vi "SDO_TRAJECTORY_EXECUTE_REL.vi"(6 "EnableClosedLoop":bool=TRUE, 8 "Init":bool, 10 "End Relative\nOrientation Deg":dbl, 11 "Gyro Heading\nRAD":dbl) -> (0 "AtReference":bool, 3 "Chassis Velocity Target":T1 {"vOmega" format="%10.3f"; "vY" format="%10.3f"; "vX" format="%10.3f"})   [LabVIEW 2019]
uses:
  <vilib>/Rock Robotics/WPI/ThirdParty/JAS_Junk/TrajLib/TypeDef/CHASSIS_SPEEDS.ctl
  <vilib>/Rock Robotics/WPI/ThirdParty/JAS_Junk/TrajLib/VI/Util_GetTime_U32.vi
  <vilib>/Rock Robotics/WPI/ThirdParty/JAS_Junk/TrajLib/ProfiledPIDController_NewPeriod.vi
  <vilib>/Rock Robotics/WPI/ThirdParty/JAS_Junk/TrajLib/ProfiledPIDController_SetIntegratorRange.vi
  <vilib>/Rock Robotics/WPI/ThirdParty/JAS_Junk/TrajLib/ProfiledPIDController_DisableContInput.vi
  <vilib>/Rock Robotics/WPI/ThirdParty/JAS_Junk/TrajLib/ProfiledPIDController_EnableContInput.vi
  <vilib>/Rock Robotics/WPI/ThirdParty/JAS_Junk/TrajLib/TrapProfConstraint_New.vi
  <vilib>/Rock Robotics/WPI/ThirdParty/JAS_Junk/TrajLib/Conv_Deg_Radians.vi
  <vilib>/Rock Robotics/WPI/ThirdParty/JAS_Junk/TrajLib/Translation2d_Create.vi
  <vilib>/Rock Robotics/WPI/ThirdParty/JAS_Junk/TrajLib/SwerveOdometry_UpdateX.vi
  <vilib>/Rock Robotics/WPI/ThirdParty/JAS_Junk/TrajLib/SwerveOdometry_ResetPosition.vi
  <vilib>/Rock Robotics/WPI/ThirdParty/JAS_Junk/TrajLib/SwerveOdometry_New.vi
  <vilib>/Rock Robotics/WPI/ThirdParty/JAS_Junk/TrajLib/HolDrvCtrl_New.vi
  <vilib>/Rock Robotics/WPI/ThirdParty/JAS_Junk/TrajLib/HolDrvCtrl_PackPID.vi
  <vilib>/Rock Robotics/WPI/ThirdParty/JAS_Junk/TrajLib/HolDrvCtrl_SetTolerance.vi
  <vilib>/Rock Robotics/WPI/ThirdParty/JAS_Junk/TrajLib/HolDrvCtrl_SetEnabled.vi
  <vilib>/Rock Robotics/WPI/ThirdParty/JAS_Junk/TrajLib/HolDrvCtrl_Calculate_Trajectory.vi
  <vilib>/Rock Robotics/WPI/ThirdParty/JAS_Junk/TrajLib/HolDrvCtrl_AtReference.vi
  <vilib>/Rock Robotics/WPI/ThirdParty/JAS_Junk/TrajLib/TrapProfState_New.vi
  <vilib>/Rock Robotics/WPI/ThirdParty/JAS_Junk/TrajLib/PIDController_NewPeriod.vi
  <vilib>/Rock Robotics/SystemInterfaces/NetworkCommunication/NetComm_UsageReport_report.vi
  <vilib>/Rock Robotics/WPI/ThirdParty/JAS_Junk/TrajLib/PIDController_SetIntegratorRange.vi
  <vilib>/Rock Robotics/WPI/ThirdParty/JAS_Junk/TrajLib/PIDController_DisableContinousInput.vi
  <vilib>/Rock Robotics/WPI/ThirdParty/JAS_Junk/TrajLib/PIDController_EnableContinousInput.vi
  <vilib>/Rock Robotics/WPI/ThirdParty/JAS_Junk/TrajLib/Rotation2d_Plus.vi
  <vilib>/Rock Robotics/WPI/ThirdParty/JAS_Junk/TrajLib/Twist2d_Create.vi
  <vilib>/Rock Robotics/WPI/ThirdParty/JAS_Junk/TrajLib/Rotation2d_Minus.vi
  <vilib>/Rock Robotics/WPI/ThirdParty/JAS_Junk/TrajLib/Pose2d_getTranslation.vi
  <vilib>/Rock Robotics/WPI/ThirdParty/JAS_Junk/TrajLib/Pose2d_New_TRRO.vi
  <vilib>/Rock Robotics/WPI/ThirdParty/JAS_Junk/TrajLib/VI/SwerveModulePosition_Get.vi
  <vilib>/Rock Robotics/WPI/ThirdParty/JAS_Junk/TrajLib/VI/SwerveModulePosition_New.vi
  <vilib>/Rock Robotics/WPI/ThirdParty/JAS_Junk/TrajLib/Twist2d_GetAll.vi
  <vilib>/Rock Robotics/WPI/ThirdParty/JAS_Junk/TrajLib/Pose2d_getRotation.vi
  <vilib>/Rock Robotics/WPI/ThirdParty/JAS_Junk/TrajLib/PIDController_Reset.vi
  <vilib>/Rock Robotics/WPI/ThirdParty/JAS_Junk/TrajLib/HolDrvCtrl_Calculate.vi
  <vilib>/Rock Robotics/WPI/ThirdParty/JAS_Junk/TrajLib/Pose2d_getXYAngle.vi
  <vilib>/Rock Robotics/WPI/ThirdParty/JAS_Junk/TrajLib/Rotation2d_GetRadians.vi
  <vilib>/Rock Robotics/WPI/ThirdParty/JAS_Junk/TrajLib/Rotation2d_RotateBy.vi
  <vilib>/Rock Robotics/WPI/ThirdParty/JAS_Junk/TrajLib/Rotation2d_UnaryMinus.vi
  <vilib>/Rock Robotics/WPI/ThirdParty/JAS_Junk/TrajLib/Rotation2d_GetAngleCosSin.vi
  <vilib>/Rock Robotics/WPI/ThirdParty/JAS_Junk/TrajLib/Pose2d_RelativeTo.vi
  <vilib>/Rock Robotics/WPI/ThirdParty/JAS_Junk/TrajLib/ProfiledPIDController_Calculate_Meas_Goal.vi
  <vilib>/Rock Robotics/WPI/ThirdParty/JAS_Junk/TrajLib/ChassisSpeeds_FromFieldRelativeSpeeds.vi
  <vilib>/Rock Robotics/WPI/ThirdParty/JAS_Junk/TrajLib/PIDController_Calculate_SP_PV.vi
  <vilib>/Rock Robotics/WPI/ThirdParty/JAS_Junk/TrajLib/ProfiledPIDController_Reset_PosOnly.vi
  <vilib>/Rock Robotics/WPI/ThirdParty/JAS_Junk/TrajLib/Rotation2d_CreateXY.vi
  <vilib>/Rock Robotics/WPI/ThirdParty/JAS_Junk/TrajLib/Transform2d_Create_PosePose.vi
  <vilib>/Rock Robotics/WPI/ThirdParty/JAS_Junk/TrajLib/ProfiledPIDController_SetGoal_PosOnly.vi
  <vilib>/Rock Robotics/WPI/ThirdParty/JAS_Junk/TrajLib/ProfiledPIDController_Calculate_Meas.vi
  <vilib>/Rock Robotics/WPI/ThirdParty/JAS_Junk/TrajLib/Rotation2d_GetCos.vi
  <vilib>/Rock Robotics/WPI/ThirdParty/JAS_Junk/TrajLib/Rotation2d_GetSin.vi
  <vilib>/Rock Robotics/WPI/ThirdParty/JAS_Junk/TrajLib/PIDController_SetSetpoint.vi
  <vilib>/Rock Robotics/WPI/ThirdParty/JAS_Junk/TrajLib/PIDController_Calculate_PV.vi
  <vilib>/Rock Robotics/WPI/ThirdParty/JAS_Junk/TrajLib/ProfiledPIDController_Reset.vi
  <vilib>/Rock Robotics/WPI/ThirdParty/JAS_Junk/TrajLib/Util_CalcDist.vi
  <vilib>/Rock Robotics/WPI/ThirdParty/JAS_Junk/TrajLib/Translation2d_Minus.vi
  <vilib>/Rock Robotics/WPI/ThirdParty/JAS_Junk/TrajLib/ProfiledPIDController_SetGoal.vi
  <vilib>/Rock Robotics/WPI/ThirdParty/JAS_Junk/TrajLib/TrapProfile_New.vi
  <vilib>/Rock Robotics/WPI/ThirdParty/JAS_Junk/TrajLib/ProfiledPIDController_GetPeriod.vi
  <vilib>/Rock Robotics/WPI/ThirdParty/JAS_Junk/TrajLib/TrapProfile_Calculate.vi
  <vilib>/Rock Robotics/WPI/ThirdParty/JAS_Junk/TrajLib/ControllerUtil_GetModulusError.vi
  <vilib>/Rock Robotics/WPI/ThirdParty/JAS_Junk/TrajLib/TrapProfile_ShouldFlipAcceleration.vi
  <vilib>/Rock Robotics/WPI/ThirdParty/JAS_Junk/TrajLib/TrapProfile_Direct.vi
  <vilib>/Rock Robotics/WPI/ThirdParty/JAS_Junk/TrajLib/PIDController_GetPeriod.vi
  Swerve_Drive_System/SDO_DRIVE_GLOBALS.vi
  <vilib>/Rock Robotics/WPI/ThirdParty/JAS_Junk/TrajLib/VI/Util_GetTime_U64.vi
  SDO_TRAJECTORY_GLOBALS.vi
  <vilib>/Rock Robotics/WPI/ThirdParty/JAS_Junk/TrajLib/Globals/Util_LibraryGlobals.vi
  <vilib>/Rock Robotics/WPI/ThirdParty/JAS_Junk/TrajLib/VI/SwerveKinematics_ToTwist2dX.vi
  <vilib>/Rock Robotics/WPI/ThirdParty/JAS_Junk/TrajLib/Pose2d_Exp.vi
  <vilib>/Rock Robotics/WPI/ThirdParty/JAS_Junk/TrajLib/Trajectory_Library.lvlib
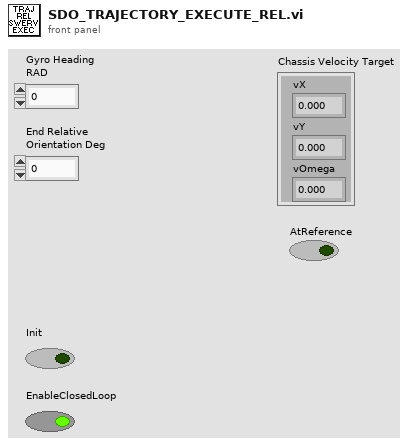
[diagram p1: front panel]
types:
  T1 = typedef "Trajectory_Library.lvlib/CHASSIS_SPEEDS.ctl" = cluster{"vX":dbl, "vY":dbl, "vOmega":dbl}
  T2 = typedef "Trajectory_Library.lvlib/ROTATION2D.ctl" = cluster{"VALUE":dbl, "COS":dbl, "SIN":dbl}
  T3 = typedef "Trajectory_Library.lvlib/SWERVE_DRIVE_KINEMATICS.ctl" = cluster{"NumModules":i32, "InverseKinematics":T4, "ForwardKinematics":T4, "Modules":T5[], "PrevCoR":T5, "SavedModuleStates":T6[]}
  T4 = typedef "NI_Matrix.lvlib/RealMatrix.ctl" = dbl[][]
  T5 = typedef "Trajectory_Library.lvlib/TRANSLATION2D.ctl" = cluster{"X":dbl, "Y":dbl}
  T6 = typedef "Trajectory_Library.lvlib/SWERVE_DRIVE_MODULE_STATE.ctl" = cluster{"Speed":dbl, "Angle":T2}
  T7 = typedef "Trajectory_Library.lvlib/SWERVE_DRIVE_MODULE_POSITION.ctl" = cluster{"Distance":dbl, "Angle":T2, "P":bool}
  T8 = typedef "Trajectory_Library.lvlib/TRAJECTORY.ctl" = cluster{"TotalTImeSecs":dbl, "States":T9[]}
  T9 = typedef "Trajectory_Library.lvlib/TRAJ_STATE.ctl" = cluster{"TimeSeconds":dbl, "Velocity":dbl, "Acceleration":dbl, "POSE":T10, "Curvature":dbl}
  T10 = typedef "Trajectory_Library.lvlib/POSE2D.ctl" = cluster{"TRANSLATION":T5, "ROTATION":T2}
  T11 = typedef "Trajectory_Library.lvlib/PID_TUNING.ctl" = cluster{"Kp":dbl, "Ki":dbl, "Kd":dbl, "MaximumIntegral":dbl, "MinimumIntegral":dbl}
  T12 = typedef "Trajectory_Library.lvlib/PROFILED_PID_CONTROLLER.ctl" = cluster{"Controller":T13, "Goal":T14, "Setpoint":T14, "Constraint":T15}
  T13 = typedef "Trajectory_Library.lvlib/PID_CONTROLLER.ctl" = cluster{"Kp":dbl, "Ki":dbl, "Kd":dbl, "Period":dbl, "Max_Integral":dbl, "Min_Integral":dbl, "Max_Input":dbl, "Min_Input":dbl, "Continuous":bool, "PositionError":dbl, "VelocityError":dbl, "PrevError":dbl, "TotalError":dbl, "PositionTolerance":dbl, "VelocityTolerance":dbl, "SetPoint":dbl, "Kf":dbl, "Prev_Deriv":dbl, "Prev_Deriv 2":dbl, "DerivativeFilter":bool, "Min_Output":dbl, "Max_Output":dbl, "Prev_F_P":dbl, "Prev_F_P_2":dbl, "AntiWindupActive":bool, "Measurement":dbl}
  T14 = typedef "Trajectory_Library.lvlib/TRAPEZOID_PROFILE_STATE.ctl" = cluster{"Position":dbl, "Velocity":dbl}
  T15 = typedef "Trajectory_Library.lvlib/TRAPEZOID_PROFILE_CONSTRAINT.ctl" = cluster{"MaxVelocity":dbl, "MaxAcceleration":dbl}
  T16 = typedef "Trajectory_Library.lvlib/HOLONOMIC_PACK_TUNING.ctl" = cluster{"X PID Tuning":T11, "Y PID Tuning":T11, "thetaProfiledPID_CTRL":T12}
  T17 = typedef "Trajectory_Library.lvlib/HOLONOMIC_DRV_CTRL.ctl" = cluster{"poseTolerance":T10, "poseError":T10, "Enabled":bool, "PID_xCtrl":T13, "PID_yCtrl":T13, "PROF_PID_thetaCtrl":T12, "RotationError":T2, "FirstRun":bool}
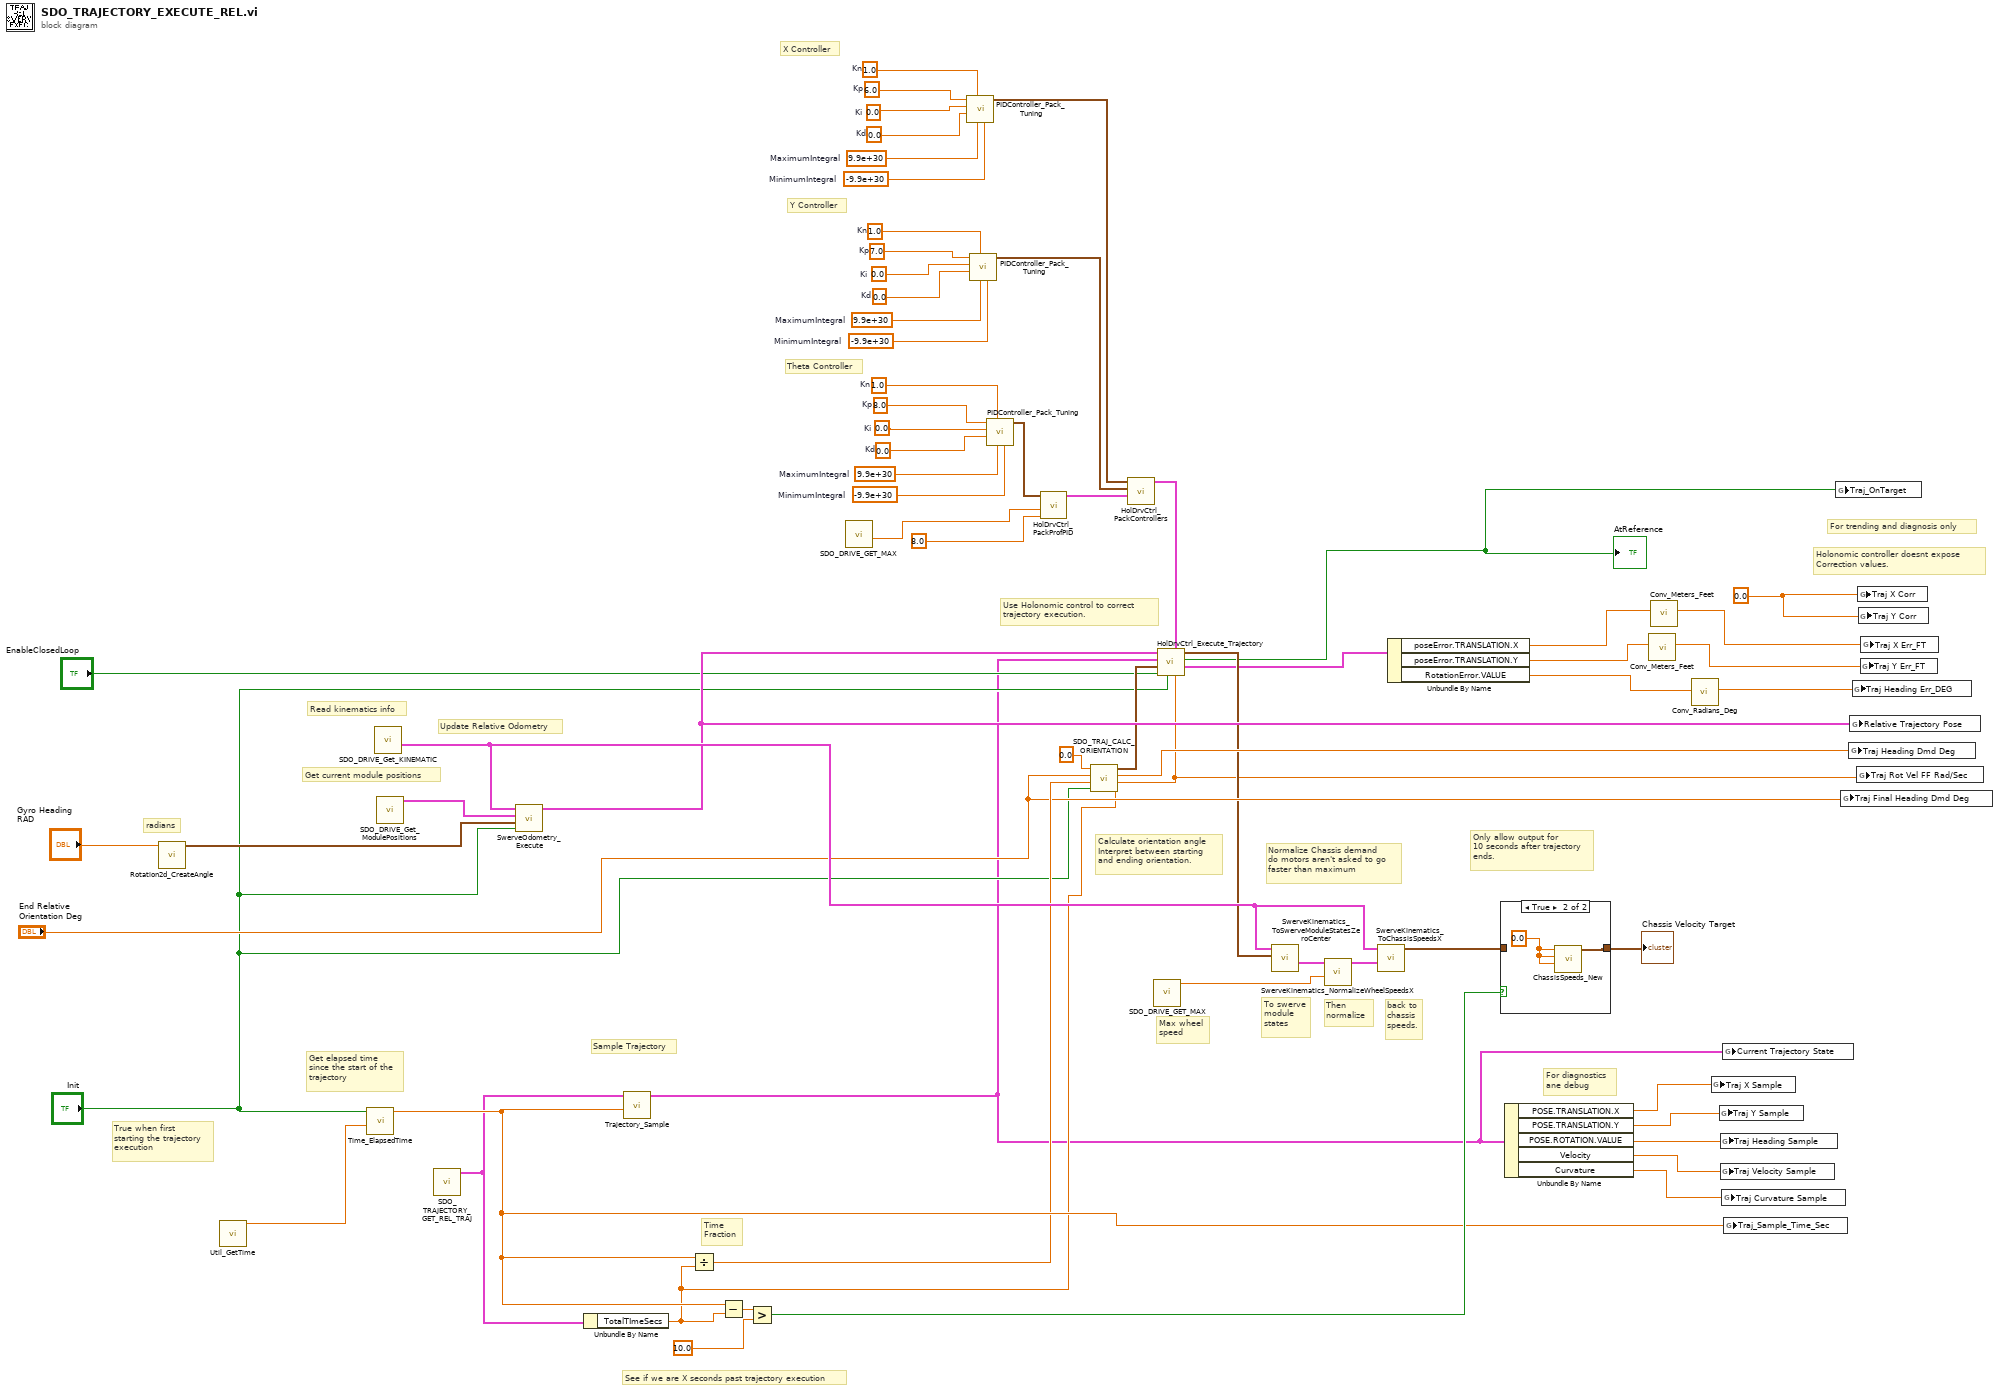
[diagram p0: block diagram]
diagram:
  w19 = 1.0  # Kn
  w22 = 8.0  # Kp
  w31 = 0.0  # Ki
  w32 = 0.0  # Kd
  w33 = 9.9e+30  # MaximumIntegral
  w34 = -9.9e+30  # MinimumIntegral
  w17 = 1.0  # Kn
  w20 = 6.0  # Kp
  w23 = 0.0  # Ki
  w24 = 0.0  # Kd
  w25 = 9.9e+30  # MaximumIntegral
  w26 = -9.9e+30  # MinimumIntegral
  w18 = 1.0  # Kn
  w21 = 7.0  # Kp
  w27 = 0.0  # Ki
  w28 = 0.0  # Kd
  w29 = 9.9e+30  # MaximumIntegral
  w30 = -9.9e+30  # MinimumIntegral
  w48 = 0.0 ("Y Corr")
  # "Theta Controller"
  # "Y Controller"
  # "X Controller"
  # "Time\nFraction"
  # "Calculate orientation angle\nInterpret between starting\nand ending orientation."
  # "Max wheel\nspeed"
  # "Get current module positions"
  # "True when first\nstarting the trajectory\nexecution"
  # "Get elapsed time\nsince the start of the\ntrajectory"
  # "Holonomic controller doesnt expose\nCorrection values."
  # "Normalize Chassis demand\ndo motors aren't asked to go\nfaster than maximum"
  # "Use Holonomic control to correct\ntrajectory execution."
  # "For trending and diagnosis only"
  # "For diagnostics\nane debug"
  # "Update Relative Odometry"
  # "back to\nchassis\nspeeds."
  # "Then\nnormalize"
  # "To swerve\nmodule\nstates"
  # "Read kinematics info"
  # "Sample Trajectory"
  # "See if we are X seconds past trajectory execution"
  # "radians"
  # "Only allow output for\n10 seconds after trajectory\nends."
  n1 = call <vilib>:"Rotation2d_CreateAngle.vi"("Angle"="Gyro Heading\nRAD") -> ("ROTATION"=w58:T2)  [unwired: 10 in]
  n2 = call <vilib>:"Util_GetTime.vi"() -> ("FPGA_Time_Seconds"=w54:dbl)  [unwired: 9 in, 2 out]
  n3 = call <vilib>:"Time_ElapsedTime.vi"("PassthroughTime_SEC"=w54, "Reset"="Init") -> ("Elapsed Time Sec"=w46:dbl)  [unwired: 9 in]
  n4 = call "SDO_DRIVE_Get_KINEMATIC.vi"() -> ("out SWERVE_DRIVE_KINEMATICS"=w56:T3)  [unwired: 11 in]
  n5 = call "SDO_DRIVE_Get_ModulePositions.vi"() -> ("Swerve Module Positions"=w55:T7[])  [unwired: 11 in]
  n6 = call "SDO_TRAJECTORY_GET_REL_TRAJ.vi"() -> ("Relative_Trajectory"=w2:T8)  [unwired: 11 in]
  n7 = call <vilib>:"SwerveOdometry_Execute.vi"("Init"="Init", "Rotation"=w58, "Swerve Module Positions"=w55, "SWERVE_DRIVE_KINEMATICS"=w56) -> ("Current Pose"=w15:T10)  [unwired: 5 in, 2 out]
  n8 = Unbundle By Name(w2) -> ("TotalTImeSecs"=w5:dbl)
  n9 = call <vilib>:"Trajectory_Sample.vi"("Time"=w46, "InputTRAJECTORY"=w2) -> ("OutputTRAJ_STATE"=w1:T9)  [unwired: 9 in]
  n10 = Divide(x=w46, y=w5) -> (x/y=w45:dbl)
  n11 = Subtract(x=w46, y=w5) -> (x-y=w66:dbl)
  n12 = Greater?(x=w66, y=10.0) -> (0:w64:bool)
  n13 = call "SDO_DRIVE_GET_MAX.vi"() -> ("Max Rotational Vel (Rad/Sec)"=w4:dbl)  [unwired: 10 in, 1 out]
  n14 = call <vilib>:"PIDController_Pack_Tuning.vi"("MinimumIntegral"=w26, "MaximumIntegral"=w25, "Kn"=w17, "Kd"=w24, "Ki"=w23, "Kp"=w20) -> ("PID Tuning"=w35:T11)  [unwired: 5 in]
  n15 = call <vilib>:"PIDController_Pack_Tuning.vi"("MinimumIntegral"=w30, "MaximumIntegral"=w29, "Kn"=w18, "Kd"=w28, "Ki"=w27, "Kp"=w21) -> ("PID Tuning"=w36:T11)  [unwired: 5 in]
  n16 = call <vilib>:"PIDController_Pack_Tuning.vi"("MinimumIntegral"=w34, "MaximumIntegral"=w33, "Kn"=w19, "Kd"=w32, "Ki"=w31, "Kp"=w22) -> ("PID Tuning"=w16:T11)  [unwired: 5 in]
  n17 = call <vilib>:"HolDrvCtrl_PackProfPID.vi"("Max Accel"=8.0, "Max Speed"=w4, "Theta PID Tuning"=w16) -> ("Theta PID CONTROLLER"=w37:T12)  [unwired: 8 in]
  n18 = call "SDO_TRAJ_CALC_ORIENTATION.vi"("Total Trajectory Time"=w5, "Init"="Init", "Time Fraction"=w45, "End Orientation Demand DEG"="End Relative\nOrientation Deg", "Starting Orientation  DEG"=0.0) -> ("Rotational Velocity"=w9:dbl, "Orientation Demand Deg"=w47:dbl, "Orientation Demand"=w14:T2)  [unwired: 4 in]
  n19 = call <vilib>:"HolDrvCtrl_PackControllers.vi"("thetaProfiledPID_CTRL"=w37, "Y PID Tuning"=w36, "X PID Tuning"=w35) -> ("HOLONOMIC_CTRL_PACK_TUNING"=w38:T16)  [unwired: 8 in]
  n20 = call "SDO_DRIVE_GET_MAX.vi"() -> ("Max Wheel Vel (Meter/Sec)"=w59:dbl)  [unwired: 10 in, 1 out]
  n21 = call <vilib>:"HolDrvCtrl_Execute_Trajectory.vi"("Rotational Velocity Feedforward \nRad/Sec"=w9, "HOLONOMIC_CTRL_PACK_TUNING"=w38, "Reset"="Init", "Enable"="EnableClosedLoop", "angleRef"=w14, "desiredTrajState"=w1, "currentPose"=w15) -> ("outHOLONOMIC_DRV_CTRL"=w11:T17, "AtReference"=w12:bool, "calcChassisSpeed"=w13:T1)  [unwired: 2 in]
  "AtReference" <- w12
  n22 = call <vilib>:"SwerveKinematics_ToSwerveModuleStatesZeroCenter.vi"("ChassisSpeeds"=w13, "in SWERVE_DRIVE_KINEMATICS"=w56) -> ("ModuleStates"=w62:T6[])  [unwired: 8 in, 1 out]
  n23 = call <vilib>:"SwerveKinematics_NormalizeWheelSpeedsX.vi"("AttainableMaxSpeed"=w59, "in WheelStates"=w62) -> ("out WheelStates"=w61:T6[])  [unwired: 9 in]
  n24 = call <vilib>:"SwerveKinematics_ToChassisSpeedsX.vi"("WheelStates"=w61, "in SWERVE_DRIVE_KINEMATICS"=w56) -> ("Chassis Speed"=w57:T1)  [unwired: 9 in]
  n25 = Unbundle By Name(w11) -> ("poseError.TRANSLATION.X"=w42:dbl, "poseError.TRANSLATION.Y"=w41:dbl, "RotationError.VALUE"=w7:dbl)
  n26 = case shown="True" w64 {
    tunnel: w57 -> [w67 _]
    tunnel: [w67 w68] -> w60
    frame False {
    }
    frame True {
      w69 = 0.0 ("vX")
      n27 = call <vilib>:"ChassisSpeeds_New.vi"("vAngular"=w69, "vY"=w69, "vX"=w69) -> ("CHASSIS"=w68:T1)  [unwired: 8 in]
    }
  }
  "Chassis Velocity Target" <- w60
  n28 = Unbundle By Name(w1) -> ("POSE.TRANSLATION.X"=w53:dbl, "POSE.TRANSLATION.Y"=w52:dbl, "POSE.ROTATION.VALUE"=w51:dbl, "Velocity"=w50:dbl, "Curvature"=w49:dbl)
  n29 = call <vilib>:"Conv_Meters_Feet.vi"("Meters"=w41) -> ("Feet"=w40:dbl)  [unwired: 10 in]
  n30 = call <vilib>:"Conv_Meters_Feet.vi"("Meters"=w42) -> ("Feet"=w39:dbl)  [unwired: 10 in]
  n31 = call <vilib>:"Conv_Radians_Deg.vi"("Radians"=w7) -> ("Degrees"=w43:dbl)  [unwired: 10 in]
  n32 = global write "SDO_TRAJECTORY_GLOBALS.vi" "Traj X Sample"(w53) -> ()
  n33 = global write "SDO_TRAJECTORY_GLOBALS.vi" "Traj Y Sample"(w52) -> ()
  n34 = global write "SDO_TRAJECTORY_GLOBALS.vi" "Traj Heading Sample"(w51) -> ()
  n35 = global write "SDO_TRAJECTORY_GLOBALS.vi" "Traj Velocity Sample"(w50) -> ()
  n36 = global write "SDO_TRAJECTORY_GLOBALS.vi" "Traj Curvature Sample"(w49) -> ()
  n37 = global write "SDO_TRAJECTORY_GLOBALS.vi" "Current Trajectory State"(w1) -> ()
  n38 = global write "SDO_TRAJECTORY_GLOBALS.vi" "Traj_Sample_Time_Sec"(w46) -> ()
  n39 = global write "SDO_TRAJECTORY_GLOBALS.vi" "Traj_OnTarget"(w12) -> ()
  n40 = global write "SDO_TRAJECTORY_GLOBALS.vi" "Traj Final Heading Dmd Deg"("End Relative\nOrientation Deg") -> ()
  n41 = global write "SDO_TRAJECTORY_GLOBALS.vi" "Traj Heading Dmd Deg"(w47) -> ()
  n42 = global write "SDO_TRAJECTORY_GLOBALS.vi" "Relative Trajectory Pose"(w15) -> ()
  n43 = global write "SDO_TRAJECTORY_GLOBALS.vi" "Traj Heading Err_DEG"(w43) -> ()
  n44 = global write "SDO_TRAJECTORY_GLOBALS.vi" "Traj Rot Vel FF Rad/Sec"(w9) -> ()
  n45 = global write "SDO_TRAJECTORY_GLOBALS.vi" "Traj X Corr"(w48) -> ()
  n46 = global write "SDO_TRAJECTORY_GLOBALS.vi" "Traj Y Corr"(w48) -> ()
  n47 = global write "SDO_TRAJECTORY_GLOBALS.vi" "Traj Y Err_FT"(w40) -> ()
  n48 = global write "SDO_TRAJECTORY_GLOBALS.vi" "Traj X Err_FT"(w39) -> ()
